vi "InitFromXML.vi"(8 "error in (no error)":errorcluster, 10 "XML":string, 11 "Web in":refnum<class "Web.lvclass">) -> (0 "error out":errorcluster, 3 "Web out":refnum<class "Web.lvclass">)   [LabVIEW 2023, in "GettingStartedWindow.lvlib" / "Web.lvclass"]
uses:
  <resource>/modes/FRC/Classes/Web/Web.lvclass
  <resource>/modes/FRC/Classes/Web/Web.lvclass/Web.ctl
  <resource>/modes/FRC/Classes/ClickableText/ClickableText.lvclass
  <resource>/modes/FRC/GettingStartedWindow.lvlib
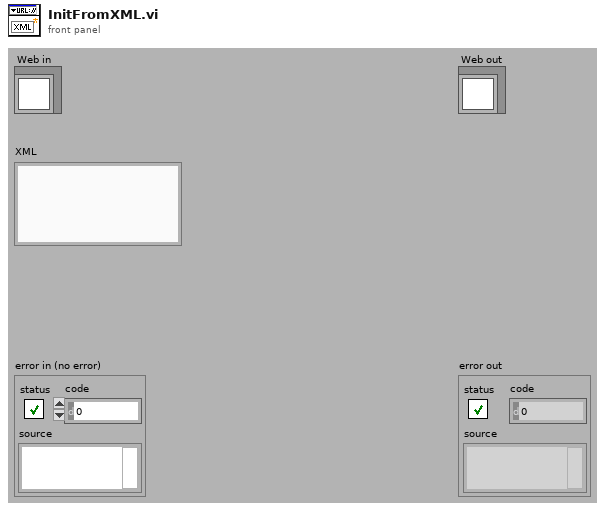
[diagram p1: front panel]
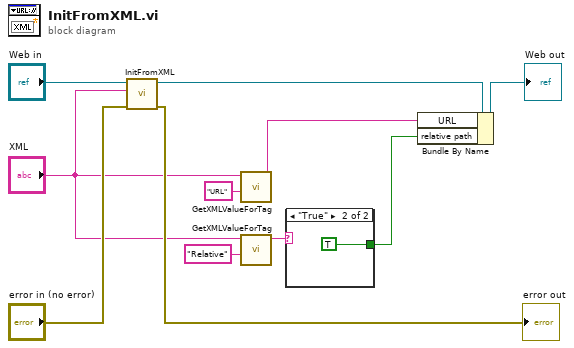
[diagram p0: block diagram]
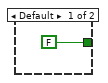
[diagram p2: hidden frame]
diagram:
  n1 = call-parent "InitFromXML.vi"("error in (no error)"="error in (no error)", "XML"="XML", "ClickableText in"="Web in") -> ("error out"=→"error out":errorcluster, "ClickableText out"=w11:refnum<class "Web.lvclass">)  [unwired: 7 out]
  n2 = call <resource>:"GetXMLValueForTag.vi"("tag"="URL", "XML"="XML") -> ("value"=w6:string)  [unwired: 1 in, 8 out]
  n3 = call <resource>:"GetXMLValueForTag.vi"("tag"="Relative", "XML"="XML") -> ("value"=w5:string)  [unwired: 1 in, 8 out]
  n4 = case shown="\"True\"" w5 {
    tunnel: [FALSE TRUE] -> w1
    frame Default {
    }
    frame "True" {
    }
  }
  n5 = Bundle By Name(cluster=w11, "URL"=w6, "relative path"=w1) -> (→"Web out":refnum<class "Web.lvclass">)
